vi "VIH Utility - STR - Add Blanks to Line Starts.vi"(10 "level":i32, 11 "String":string) -> (3 "String out":string)   [LabVIEW 2014]
doc: "::: VI Helpeks :::\nCopyright (c) 2000-2026 Konstantin Shifershteyn. All rights reserved."
panel:
  in  "blanks (2)":i32=2
  in  "blank char (\\s)":string=" "
  # "VI Helpeks\nCopyright (c) 2012-2026 Konstantin Shifershteyn"
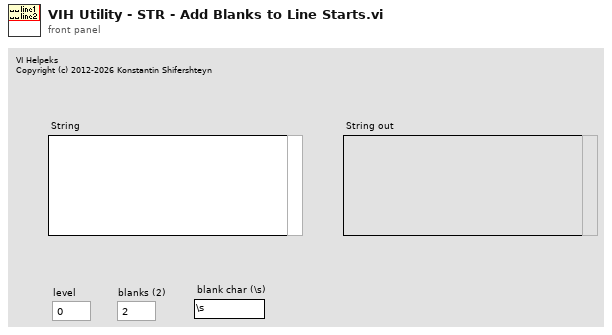
[diagram p1: front panel]
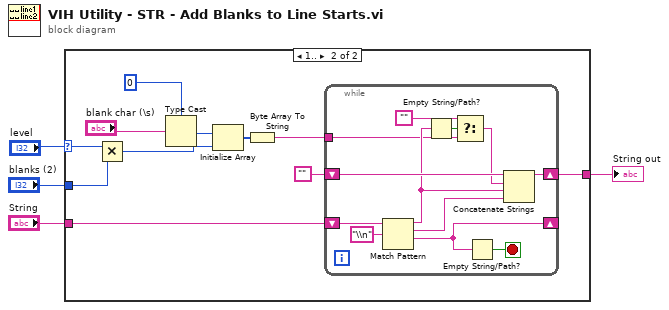
[diagram p0: block diagram]
diagram:
  n1 = case shown="1.." "level" {
    selector: "level" -> [_ w8]
    tunnel: "String" -> [w5 w12]
    tunnel: [w5 w9] -> w2
    tunnel: "blanks (2)" -> [_ w7]
    frame ..0 {
    }
    frame 1.. {
      n2 = Multiply(x=w8, y=w7) -> (x*y=w6:i32)
      n3 = Type Cast(type=u8 0, x="blank char (\\s)") -> (*(type *) &x=w13:u8)
      n4 = Initialize Array(w13, w6) -> (w16:u8[])
      n5 = Byte Array To String(unsigned byte array=w16) -> (string=w10:string)
      n6 = while {
        shift-right: [w26] -> _
        shift-left: w12 -> [w28]
        shift-right: [w17] -> w9
        shift-left: "" -> [w24]
        tunnel: w10 -> [w20]
        stop <- w25 stop-if-true
        n7 = Match Pattern(string=w28, regular expression="\\n") -> (before substring=w22:string, match substring=w23:string, after substring=w26:string)  [unwired: 1 in, 1 out]
        n8 = Empty String/Path?(string/path=w22) -> (empty?=w21:bool)
        n9 = Select(t="", s=w21, f=w20) -> (s? t:f=w18:string)
        n10 = Empty String/Path?(string/path=w26) -> (empty?=w25:bool)
        n11 = Concatenate Strings(w24, w18, w22, w23) -> (w17:string)
      }
    }
  }
  "String out" <- w2
